vi "PicoScope6000SetupStreaming.vi"(0 "handle in":i16, 1 "Device Info":T2, 3 "Acquisition Settings":T3 {"Time Units" items=["Nanoseconds (ns)", "Microseconds (us)", "Milliseconds (ms)", "Seconds (s)"]; "Down-Sample Mode" items=["None", "Aggregate", "Decimate", "Average"]}, 4 "Buffer and Transfer Settings":T1 {"Down-Sample Mode" items=["None", "Aggregate", "Decimate", "Average"]; "Down Sample Ratio" step=1; "Samples" format="%_6p"}, 5 "error in":errorcluster, 8 "enabled array":i16[](array[numeric]), 10 "Pointers In":u64[][](array[numeric])) -> (11 "Pointer array":u64[][](array[numeric]), 14 "handle out":i16, 16 "sampleIntervalTimeUnits":u32, 17 "Sample Interval":u32, 19 "error out":errorcluster)   [LabVIEW 2009]
doc: "Set up the data buffers and calls RunStreaming to start the device streaming.\nData will be copied from the driver buffers into the corresponding application buffers using the wrapper dll."
uses:
  ps6000Wrap.dll
  ps6000.dll
panel:
  # "Overview Buffer Size is the size of the temporary buffers used to\nstore data before returning it to the application."
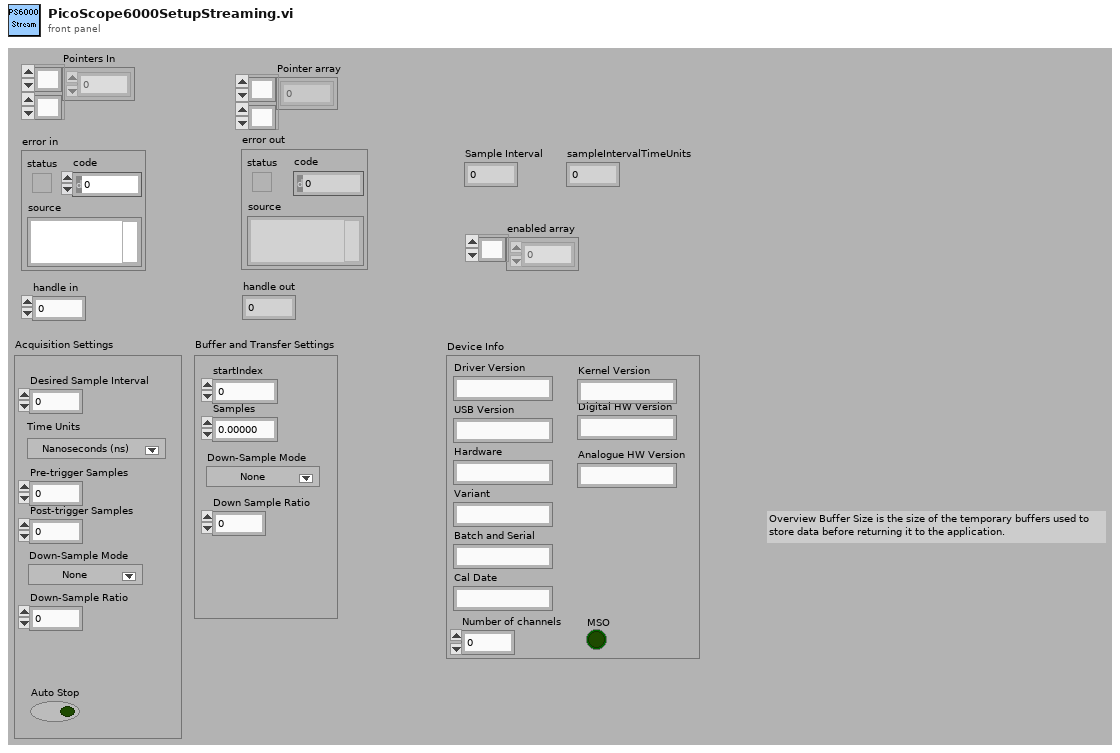
[diagram p1: front panel]
types:
  T1 = cluster{"startIndex":u64, "Samples":u64, "Down Sample Ratio":u64, "Down-Sample Mode":u32}
  T2 = cluster{"Driver Version":string, "USB Version":string, "Hardware":string, "Variant":string, "Batch and Serial":string, "Cal Date":string, "Kernel Version":string, "Digital HW Version":string, "Analogue HW Version":string, "MSO":bool, "Number of channels":i16}
  T3 = cluster{"Auto Stop":bool, "Desired Sample Interval":u32, "Pre-trigger Samples":u32, "Post-trigger Samples":u32, "Down-Sample Ratio":u32, "Down-Sample Mode":i32, "Time Units":u32}
  T4 = cluster{"status":bool, "code":u32, "source":string}
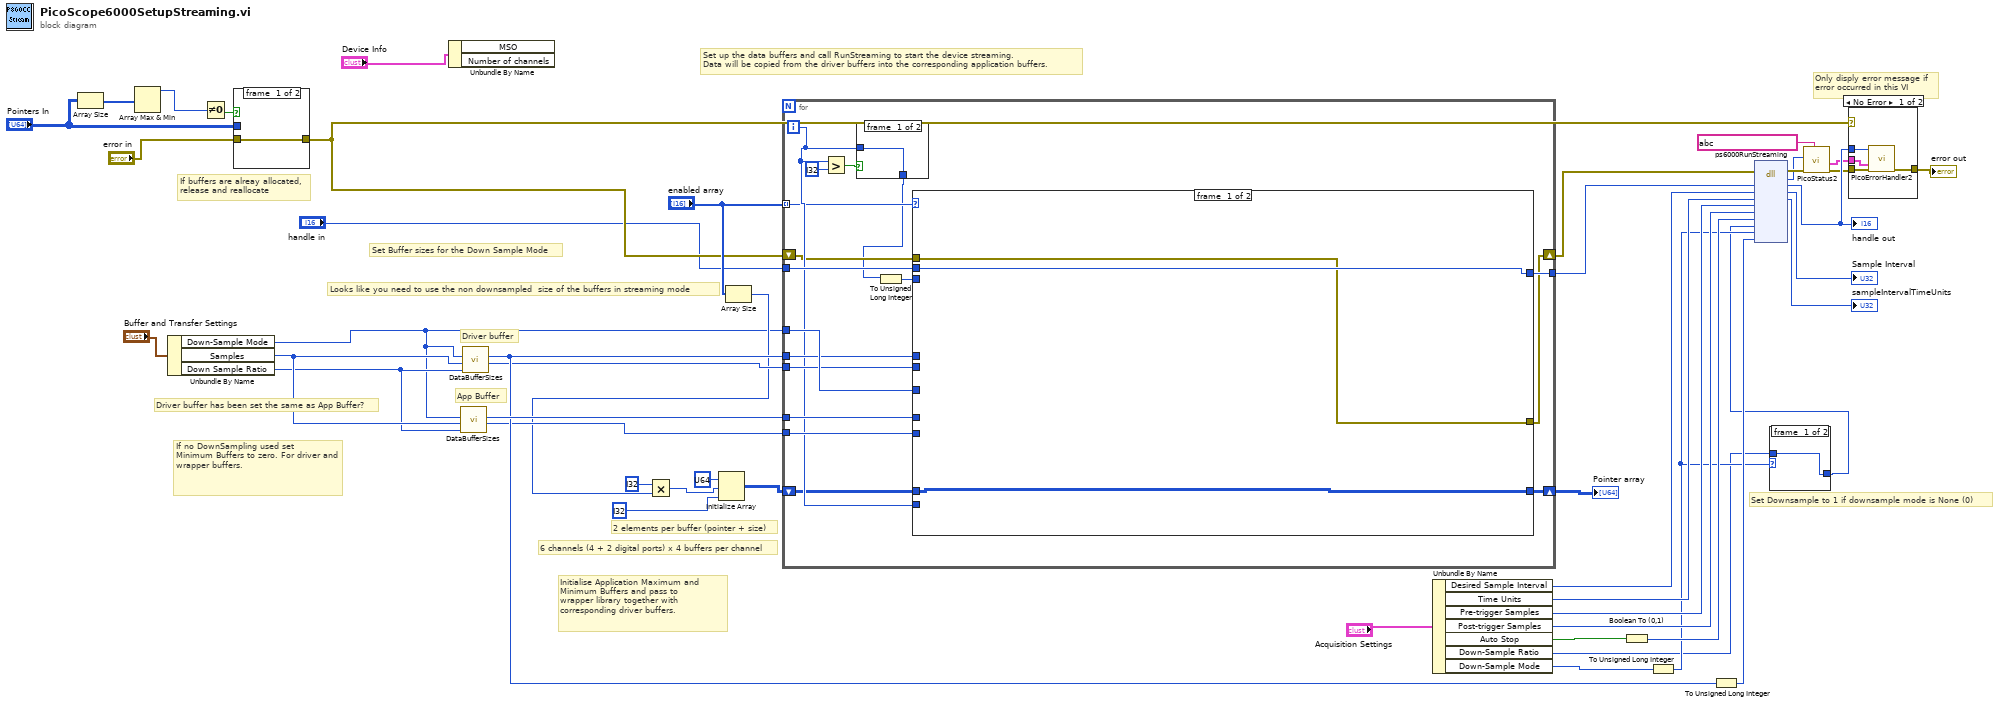
[diagram p0: block diagram]
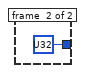
[diagram p2: hidden frame]
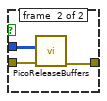
[diagram p3: hidden frame]
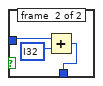
[diagram p4: hidden frame]
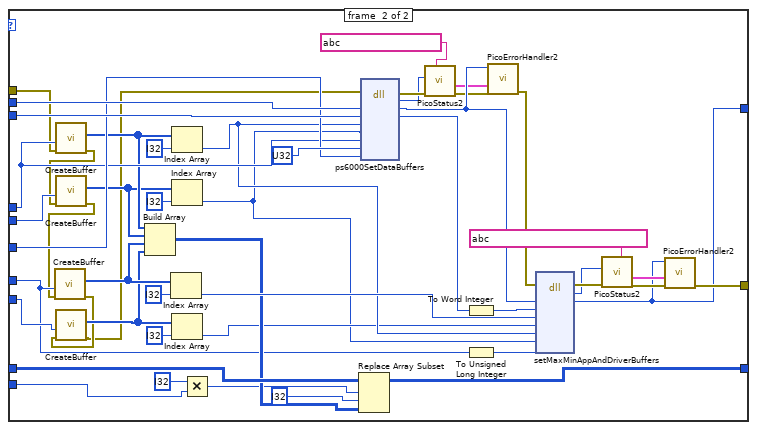
[diagram p5: hidden frame]
diagram:
  # "Set Downsample to 1 if downsample mode is None (0)"
  # "Looks like you need to use the non downsampled  size of the buffers in streaming mode"
  # "If buffers are alreay allocated,\nrelease and reallocate"
  # "2 elements per buffer (pointer + size)"
  # "6 channels (4 + 2 digital ports) x 4 buffers per channel"
  # "App Buffer"
  # "Driver buffer"
  # "Driver buffer has been set the same as App Buffer?"
  # "Set Buffer sizes for the Down Sample Mode"
  # "If no DownSampling used set \nMinimum Buffers to zero. For driver and wrapper buffers."
  # "Initialise Application Maximum and\nMinimum Buffers and pass to \nwrapper library together with corresponding driver buffers."
  # "Only disply error message if\nerror occurred in this VI"
  # "Set up the data buffers and call RunStreaming to start the device streaming.\nData will be copied from the driver buffers into the corresponding application buffers."
  n1 = Array Size(array="Pointers In") -> (size(s)=w14:i32[])
  n2 = Array Max & Min(array=w14) -> (max value=w13:i32)  [unwired: 3 out]
  n3 = Unbundle By Name("Buffer and Transfer Settings") -> ("Down-Sample Mode"=w11:u32, "Samples"=w35:u64, "Down Sample Ratio"=w34:u64)
  n4 = Not Equal To 0?(x=w13) -> (x != 0?=w19:bool)
  n5 = case shown="True" w19 {
    tunnel: "Pointers In" -> [_ w49]
    tunnel: "error in" -> [w48 w50]
    tunnel: [w48 w51] -> w7
    frame #0 {
    }
    frame #1 {
      n6 = call "PicoReleaseBuffers.vi"("error in (no error)"=w50, "Pointer array"=w49) -> ("error out"=w51:errorcluster)  [unwired: 8 in, 1 out]
    }
  }
  n7 = Unbundle By Name("Device Info") -> ()  [unwired: 2 out]
  n8 = call "DataBufferSizes.vi"("Down Sample Ratio"=w34, "Number of Samples"=w35, "Down-Sample Mode"=w11) -> ("min Buffer Size"=w30:i32, "Max Buffer Size"=w33:i32)  [unwired: 7 in]
  n9 = call "DataBufferSizes.vi"("Down Sample Ratio"=w34, "Number of Samples"=w35, "Down-Sample Mode"=w11) -> ("min Buffer Size"=w31:i32, "Max Buffer Size"=w32:i32)  [unwired: 7 in]
  n10 = Array Size(array="enabled array") -> (size(s)=w23:i32)
  n11 = Multiply(x=i32 ?, y=w23) -> (x*y=w24:i32)
  n12 = Initialize Array(u64 ? ("element"), w24, i32 ? ("dimension size")) -> (w15:u64[][])
  n13 = for {
    tunnel: "enabled array" -> [w57] mode=indexing
    tunnel: "handle in" -> [w68]
    tunnel: w11 -> [w67]
    tunnel: w33 -> [w66]
    tunnel: w32 -> [w65]
    tunnel: w31 -> [w64]
    tunnel: w30 -> [w63]
    tunnel: [w58] -> w26
    shift-right: [w56] -> w20
    shift-left: w7 -> [w55]
    shift-right: [w62] -> w29
    shift-left: w15 -> [w54]
    i -> [w59]
    n14 = Greater?(x=w59, y=i32 ?) -> (0:w60:bool)
    n15 = case shown="True" w60 {
      tunnel: [w69 w70] -> w52
      tunnel: w59 -> [w69 w72]
      frame #0 {
      }
      frame #1 {
        n16 = Add(x=w72, y=i32 ?) -> (x+y=w70:i32)
      }
    }
    n17 = To Unsigned Long Integer(number=w52) -> (unsigned 32bit integer=w53:u32)
    n18 = case shown="1" w57 {
      tunnel: w68 -> [w74 w124]
      tunnel: w55 -> [w73 w92]
      tunnel: w53 -> [_ w120]
      tunnel: w66 -> [_ w95]
      tunnel: w65 -> [_ w112]
      tunnel: w64 -> [_ w115]
      tunnel: w63 -> [_ w114]
      tunnel: w67 -> [_ w113]
      tunnel: w54 -> [w75 w106]
      tunnel: [w75 w105] -> w62
      tunnel: w59 -> [_ w102]
      tunnel: [w74 w76] -> w58
      tunnel: [w73 w78] -> w56
      frame #0 {
      }
      frame #1 {
        n19 = call "CreateBuffer.vi"("error in (no error)"=w92, "Buffer size"=w112) -> ("error out"=w91:errorcluster, "Pointer and BufferSize"=w110:u64[])  [unwired: 8 in]
        n20 = call "CreateBuffer.vi"("error in (no error)"=w91, "Buffer size"=w115) -> ("error out"=w90:errorcluster, "Pointer and BufferSize"=w109:u64[])  [unwired: 8 in]
        n21 = call "CreateBuffer.vi"("error in (no error)"=w90, "Buffer size"=w95) -> ("error out"=w89:errorcluster, "Pointer and BufferSize"=w108:u64[])  [unwired: 8 in]
        n22 = call "CreateBuffer.vi"("error in (no error)"=w89, "Buffer size"=w114) -> ("error out"=w88:errorcluster, "Pointer and BufferSize"=w107:u64[])  [unwired: 8 in]
        n23 = Build Array(w110, w109, w108, w107) -> (w101:u64[][])
        n24 = Index Array(array=w108, index=i32 ?) -> (element=w111:u64)
        n25 = Index Array(array=w110, index=i32 ?) -> (element=w104:u64)
        n26 = Index Array(array=w109, index=i32 ?) -> (element=w93:u64)
        n27 = Index Array(array=w107, index=i32 ?) -> (element=w94:u64)
        n28 = Multiply(x=i32 ?, y=w102) -> (x*y=w100:i32)
        n29 = Replace Array Subset(array=w106, new element=w101, index (row)=w100, index (col)=i32 ? ("disabled index (row)")) -> (w105:u64[][])
        n30 = dll-call lib="ps6000.dll" fn="ps6000SetDataBuffers" ("ps3000.dll:_ps3000_open_unit@0")(error in=w88, "handle"=w124, "channel"=w120, "bufferMax"=w104, "bufferMin"=w93, "bufferLth"=w112, "segmentIndex"=u32 ?, "downSampleRatioMode"=w113) -> (error out=w86:errorcluster, "PICO_STATUS"=w85:u32, "handle"=w97:i16, "channel"=w121:u32)  [unwired: 7 in, 1 out]
        n31 = call "PicoStatus2.vi"("PICO source"=string ? ("source"), "Error in"=w86, "PICO STATUS"=w85) -> ("error out"=w87:errorcluster, "PICO_STATUS out"=w83:T4)  [unwired: 5 in]
        n32 = To Word Integer(number=w121) -> (16bit integer=w122:i16)
        n33 = To Unsigned Long Integer(number=w95) -> (unsigned 32bit integer=w96:u32)
        n34 = call "PicoErrorHandler2.vi"("error in (no error)"=w87, "PICO_STATUS in"=w83, "handle In"=w97) -> ("error out"=w98:errorcluster)  [unwired: 8 in]
        n35 = dll-call lib="ps6000Wrap.dll" fn="setMaxMinAppAndDriverBuffers"(error in=w98, "handle"=w97, "channel"=w122, "appMaxBuffer"=w111, "appMinBuffer"=w94, "driverMaxBuffer"=w104, "driverMinBuffer"=w93, "bufferLength"=w96) -> (error out=w82:errorcluster, "status"=w81:i16, "handle"=w76:i16)  [unwired: 8 in, 1 out]
        n36 = call "PicoStatus2.vi"("PICO source"=string ? ("source"), "Error in"=w82, "PICO STATUS"=w81) -> ("error out"=w79:errorcluster, "PICO_STATUS out"=w77:T4)  [unwired: 5 in]
        n37 = call "PicoErrorHandler2.vi"("error in (no error)"=w79, "PICO_STATUS in"=w77, "handle In"=w76) -> ("error out"=w78:errorcluster)  [unwired: 8 in]
      }
    }
  }
  "Pointer array" <- w29
  n38 = Unbundle By Name("Acquisition Settings") -> ("Desired Sample Interval"=w44:u32, "Time Units"=w38:u32, "Pre-trigger Samples"=w43:u32, "Post-trigger Samples"=w42:u32, "Auto Stop"=w41:bool, "Down-Sample Ratio"=w9:u32, "Down-Sample Mode"=w39:i32)
  n39 = Boolean To (0,1)(Boolean=w41) -> (0, 1=w45:i16)
  n40 = To Unsigned Long Integer(number=w39) -> (unsigned 32bit integer=w10:u32)
  n41 = To Unsigned Long Integer(number=w32) -> (unsigned 32bit integer=w12:u32)
  n42 = case shown="0" w10 {
    tunnel: [w125 u32 ? ("Down-Sample Ratio")] -> w8
    tunnel: w9 -> [w125 _]
    frame #0 {
    }
    frame #1 {
    }
  }
  n43 = dll-call lib="ps6000.dll" fn="ps6000RunStreaming" ("ps5000a.dll:_ps3000_open_unit@0")(error in=w20, "handle"=w26, "sampleInterval"=w44, "sampleIntervalTimeUnits"=w38, "maxPreTriggerSamples"=w43, "maxPostTriggerSamples"=w42, "autoStop"=w45, "downSampleRatio"=w8, "downSampleRatioMode"=w10, "overviewBufferSize"=w12) -> (error out=w5:errorcluster, "PICO_STATUS"=w4:u32, "handle"=w16:i16, "sampleInterval"=→"Sample Interval":u32, "sampleIntervalTimeUnits"=→"sampleIntervalTimeUnits":u32)  [unwired: 8 in, 1 out]
  "handle out" <- w16
  n44 = call "PicoStatus2.vi"("PICO source"=string ? ("source"), "Error in"=w5, "PICO STATUS"=w4) -> ("error out"=w2:errorcluster, "PICO_STATUS out"=w1:T4)  [unwired: 5 in]
  n45 = case shown="No Error" w7 {
    tunnel: [w129 w131] -> w47
    tunnel: w2 -> [w130 w131]
    tunnel: w16 -> [w128 _]
    tunnel: w1 -> [w127 _]
    frame #0 {
      n46 = call "PicoErrorHandler2.vi"("error in (no error)"=w130, "PICO_STATUS in"=w127, "handle In"=w128) -> ("error out"=w129:errorcluster)  [unwired: 8 in]
    }
    frame #1 {
    }
  }
  "error out" <- w47
